vi "Logging Message Loop.vi"(8 "error in (no error)":errorcluster, 10 "Data Queue":refnum<queue>, 11 "Message Queues":T1) -> (0 "error out":errorcluster)   [LabVIEW 2021, in "Logging.lvlib"]
doc: "Message loop for handling messages pertaining to logging data."
uses:
  Logging.lvlib
  support/Message Queue/All Message Queues.ctl
  support/Message Queue/Message Cluster.ctl
  Acquisition/Acquired Data.ctl
  Logging State.ctl
  support/Message Queue/Enqueue Message (Single).vi
  <vilib>/Utility/error.llb/Error Cluster From Error Code.vi
  <vilib>/ErrorRing/Error Ring.xnode
  support/Message Queue/Message Queue.lvlib
  Settings/Settings.lvlib
  Acquisition/Acquisition.lvlib
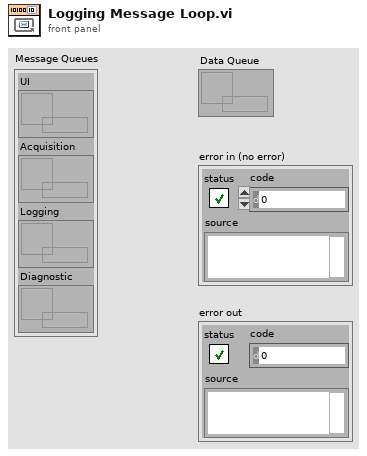
[diagram p1: front panel]
types:
  T1 = typedef "Message Queue.lvlib/All Message Queues.ctl" = cluster{"UI":refnum<queue>, "Acquisition":refnum<queue>, "Logging":refnum<queue>, "Diagnostic":refnum<queue>}
  T2 = typedef "Logging.lvlib/Logging State.ctl" = enum16{"Idle", "Logging"}
  T3 = typedef "Settings.lvlib/Settings.ctl" = cluster{"IO":T4, "Log":T11, "Debug":T13}
  T4 = typedef "Acquisition.lvlib/Hardware Configuration.ctl" = cluster{"Channel Settings":T5[], "Sensor Intervals":T7[], "Sensor Token":T9, "API":T10}
  T5 = typedef "Acquisition.lvlib/Channel Settings.ctl" = cluster{"Name":string, "Terminal Information":cluster{"IO Device":T6, "Channel Number":i32}, "Calibration Information":cluster{"Excitation Voltage":dbl, "Calibration Factor":dbl, "Zero Value":dbl, "Calibration Formula":string}}
  T6 = typedef "Acquisition.lvlib/IO Device.ctl" = enum16{"none", "9219", "9401"}
  T7 = typedef "Interval Timer.lvlib/Repeat Interval.ctl" = cluster{"Interval":T8, "Count":i32}
  T8 = typedef "Interval Timer.lvlib/Interval Length.ctl" = enum16{"Manual control", "1 second", "10 seconds", "30 seconds", "60 seconds", "600 seconds", "1200 seconds", "3600 seconds"}
  T9 = typedef "Interval Timer.lvlib/Interval Token.ctl" = cluster{"Next reading in ms":u32, "Interval Index":i32, "Interval Occurrence":i32}
  T10 = typedef "Acquisition.lvlib/IO API.ctl" = enum16{"Simulated", "DAQmx"}
  T11 = typedef "Logging.lvlib/Logging Configuration.ctl" = cluster{"Path":path, "Spreadsheet":refnum<file>, "Mode":T12}
  T12 = typedef "Logging.lvlib/Logging Mode.ctl" = enum16{"Overwrite", "Append", "Create New"}
  T13 = typedef "Diagnostics.lvlib/Diagnostics Configuration.ctl" = cluster{"Messages":refnum<file>}
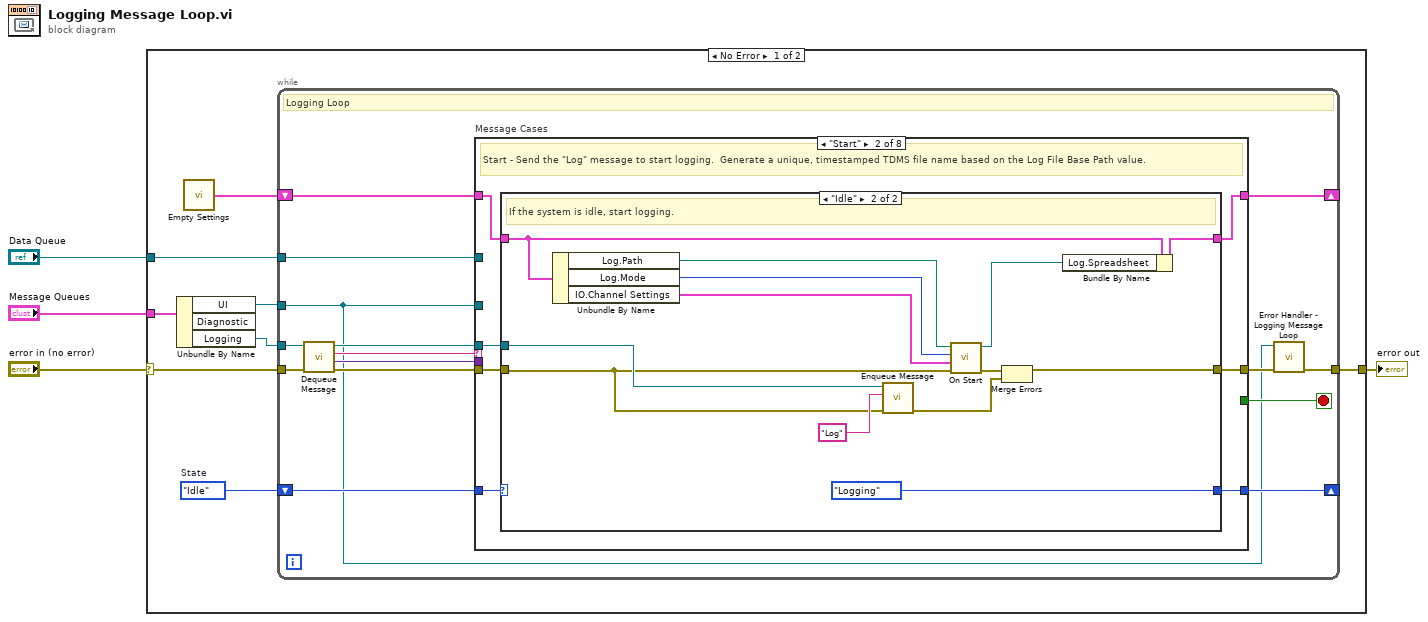
[diagram p0: block diagram]
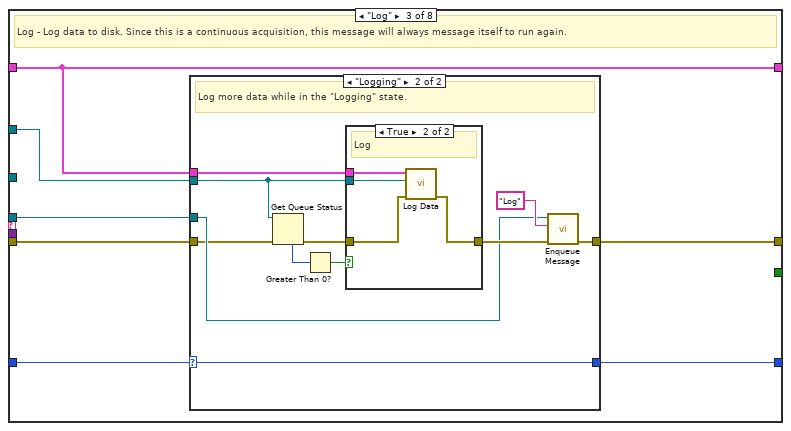
[diagram p4: hidden frame]
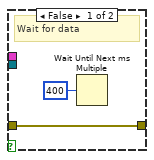
[diagram p6: hidden frame]
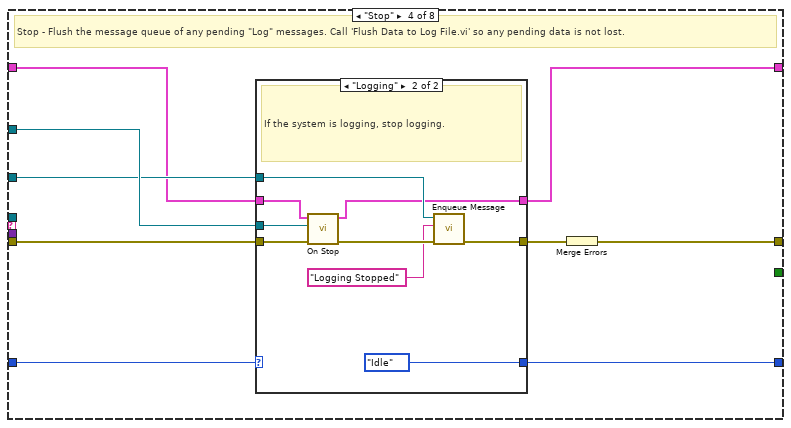
[diagram p7: hidden frame]
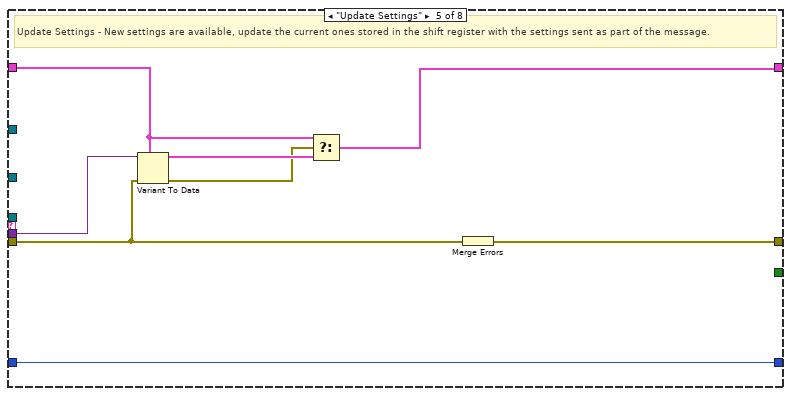
[diagram p9: hidden frame]
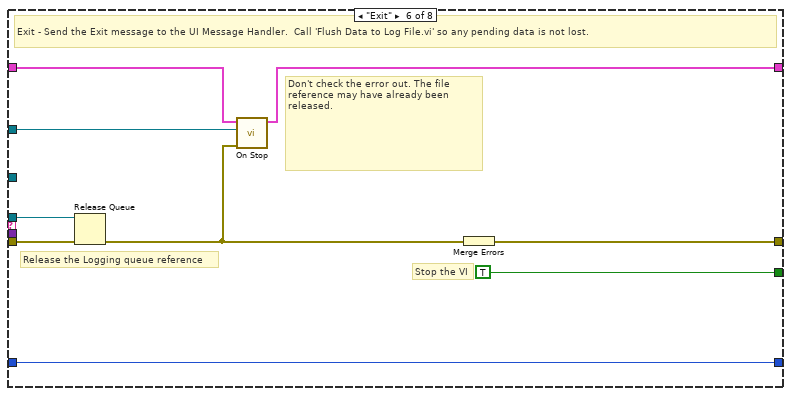
[diagram p10: hidden frame]
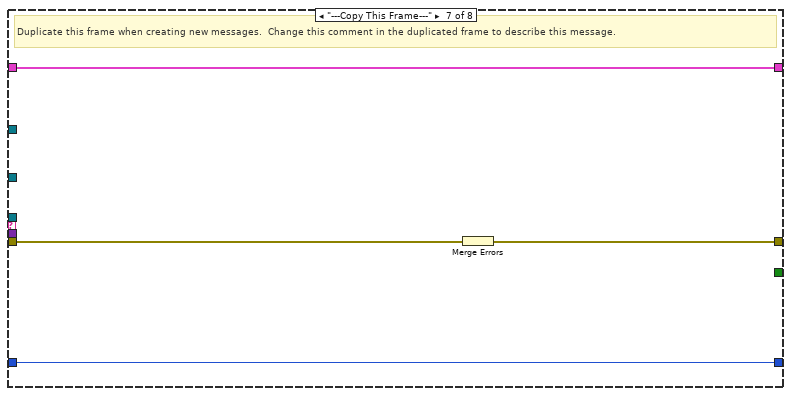
[diagram p11: hidden frame]
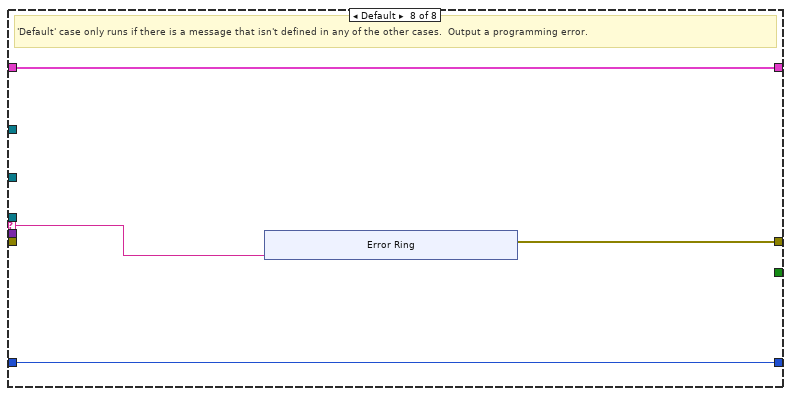
[diagram p12: hidden frame]
diagram:
  n1 = case shown="No Error" "error in (no error)" {
    selector: "error in (no error)" -> [w10 w133]
    tunnel: "Message Queues" -> [w12 _]
    tunnel: [w11 w133] -> w3
    tunnel: "Data Queue" -> [w9 _]
    frame No Error {
      w7 = Logging_State."Idle"  # State
      n2 = Unbundle By Name(w12) -> ("UI"=w8:refnum<queue>, "Logging"=w5:refnum<queue>)  [unwired: 1 out]
      n3 = call "Empty Settings.vi"() -> ("Settings"=w6:T3)
      n4 = while {
        tunnel: w5 -> [w19]
        shift-right: [w26] -> _
        shift-left: w6 -> [w27]
        tunnel: w8 -> [w13]
        tunnel: w9 -> [w18]
        shift-right: [w16] -> _
        shift-left: w7 -> [w17]
        tunnel: w10 -> [w24]
        tunnel: [w15] -> w11
        stop <- w25 stop-if-true
        # "Logging Loop"
        n5 = call "Dequeue Message.vi"("error in (no error)"=w24, "Message Queue"=w19) -> ("error out"=w23:errorcluster, "Message Data"=w21:variant, "Message"=w22:string, "dup Message Queue"=w20:refnum<queue>)  [unwired: 6 in]
        n6 = case "Message Cases" shown="\"Start\"" w22 {
          selector: w22 -> [_ _ _ _ _ _ _ w122]
          tunnel: w20 -> [_ w36 w59 _ _ w114 _ _]
          tunnel: w23 -> [w29 w35 w57 w85 w102 w115 w121 _]
          tunnel: [w29 w37 w60 w88 w108 w116 w119 w123] -> w14
          tunnel: w27 -> [w30 w34 w56 w80 w106 w110 w120 w125]
          tunnel: [w30 w33 w56 w81 w103 w109 w120 w125] -> w26
          tunnel: [_ _ _ _ _ TRUE _ _] -> w25
          tunnel: w21 -> [_ _ _ _ w107 _ _ _]
          tunnel: w13 -> [_ _ _ w82 _ _ _ _]
          tunnel: w18 -> [_ _ w58 w86 _ w112 _ _]
          tunnel: w17 -> [w28 w32 w55 w84 w101 w111 w118 w124]
          tunnel: [w28 w31 w54 w83 w101 w111 w118 w124] -> w16
          frame "Initialize" {
            # "Initialize - gets called when first launched. Currently a no-op."
          }
          frame "Start" {
            # "Start - Send the \"Log\" message to start logging.  Generate a unique, timestamped TDMS file name based on the Log File Base Path value."
            n7 = case shown="\"Idle\"" w32 {
              selector: w32 -> [w39 _]
              tunnel: [w38 w47] -> w37
              tunnel: w36 -> [_ w48]
              tunnel: w35 -> [w38 w46]
              tunnel: w34 -> [w40 w49]
              tunnel: [w40 w51] -> w33
              tunnel: [w39 Logging_State."Logging" ("State")] -> w31
              frame "Logging" {
                # "The system is already logging. Ignore the \"Start\" message."
              }
              frame "Idle" {
                # "If the system is idle, start logging."
                n8 = Unbundle By Name(w49) -> ("Log.Path"=w43:path, "Log.Mode"=w44:T12, "IO.Channel Settings"=w41:T5[])
                n9 = call-poly "Enqueue Message.vi"("error in (no error)"=w46, "Message"="Log", "Message Queue"=w48) -> ("error out"=w52:errorcluster)  [unwired: 7 in, 1 out]
                n10 = call "On Start.vi"("error in"=w46, "Channel Settings"=w41, "Mode"=w44, "file path"=w43) -> ("error out"=w45:errorcluster, "file reference"=w42:refnum<file>)  [unwired: 6 in]
                n11 = Merge Errors(w45, w52) -> (w47:errorcluster)
                n12 = Bundle By Name(cluster=w49, "Log.Spreadsheet"=w42) -> (w51:T3)
              }
            }
          }
          frame "Log" {
            # "Log - Log data to disk. Since this is a continuous acquisition, this message will always message itself to run again."
            n13 = case shown="\"Logging\"" w55 {
              selector: w55 -> [w62 w71]
              tunnel: [w61 w70] -> w60
              tunnel: w59 -> [_ w68]
              tunnel: w58 -> [_ w65]
              tunnel: w57 -> [w61 w67]
              tunnel: w56 -> [_ w72]
              tunnel: [w62 w71] -> w54
              frame "Idle" {
                # "Ignore \"Log\" messages when the logging is idle."
              }
              frame "Logging" {
                # "Log more data while in the \"Logging\" state."
                n14 = Get Queue Status(queue=w65, error in (no error)=w67) -> (error out=w66:errorcluster, # elements in queue=w64:i32)  [unwired: 1 in, 6 out]
                n15 = Greater Than 0?(x=w64) -> (x > 0?=w63:bool)
                n16 = case shown="True" w63 {
                  tunnel: w65 -> [_ w79]
                  tunnel: w72 -> [_ w78]
                  tunnel: w66 -> [w75 w77]
                  tunnel: [w75 w76] -> w69
                  frame False {
                    # "Wait for data"
                    n17 = Wait Until Next ms Multiple(millisecond multiple=u32 400) -> ()  [unwired: 1 out]
                  }
                  frame True {
                    # "Log"
                    n18 = call "Log Data.vi"("error in (no error)"=w77, "Data Queue"=w79, "Settings"=w78) -> ("error out"=w76:errorcluster)  [unwired: 8 in]
                  }
                }
                n19 = call-poly "Enqueue Message.vi"("error in (no error)"=w69, "Message"="Log", "Message Queue"=w68) -> ("error out"=w70:errorcluster)  [unwired: 7 in, 1 out]
              }
            }
          }
          frame "Stop" {
            # "Stop - Flush the message queue of any pending \"Log\" messages. Call 'Flush Data to Log File.vi' so any pending data is not lost."
            n20 = case shown="\"Logging\"" w84 {
              selector: w84 -> [w90 _]
              tunnel: [w91 w95] -> w87
              tunnel: w86 -> [_ w99]
              tunnel: w80 -> [w89 w98]
              tunnel: w85 -> [w91 w97]
              tunnel: [w90 Logging_State."Idle" ("State")] -> w83
              tunnel: w82 -> [_ w94]
              tunnel: [w89 w92] -> w81
              frame "Idle" {
                # "The system is already idle. Ignore the \"Stop\" message."
              }
              frame "Logging" {
                # "If the system is logging, stop logging."
                n21 = call "On Stop.vi"("error in (no error)"=w97, "Data Queue"=w99, "Settings in"=w98) -> ("error out"=w100:errorcluster, "Settings out"=w92:T3)  [unwired: 7 in]
                n22 = call-poly "Enqueue Message.vi"("error in (no error)"=w100, "Message"="Logging Stopped", "Message Queue"=w94) -> ("error out"=w95:errorcluster)  [unwired: 7 in, 1 out]
              }
            }
            n23 = Merge Errors(w87) -> (w88:errorcluster)
          }
          frame "Update Settings" {
            # "Update Settings - New settings are available, update the current ones stored in the shift register with the settings sent as part of the message."
            n24 = Variant To Data(error in=w102, type=w106, Variant=w107) -> (data=w105:T3, error out=w104:errorcluster)
            n25 = Select(t=w106, s=w104, f=w105) -> (s? t:f=w103:T3)
            n26 = Merge Errors(w102) -> (w108:errorcluster)
          }
          frame "Exit" {
            # "Don't check the error out. The file reference may have already been released."
            # "Release the Logging queue reference"
            # "Stop the VI"
            # "Exit - Send the Exit message to the UI Message Handler.  Call 'Flush Data to Log File.vi' so any pending data is not lost."
            n27 = Release Queue(queue=w114, error in (no error)=w115) -> (error out=w113:errorcluster)  [unwired: 1 in, 2 out]
            n28 = call "On Stop.vi"("error in (no error)"=w113, "Data Queue"=w112, "Settings in"=w110) -> ("Settings out"=w109:T3)  [unwired: 7 in, 1 out]
            n29 = Merge Errors(w113) -> (w116:errorcluster)
          }
          frame "---Copy This Frame---" {
            # "Duplicate this frame when creating new messages.  Change this comment in the duplicated frame to describe this message."
            n30 = Merge Errors(w121) -> (w119:errorcluster)
          }
          frame Default {
            # "'Default' case only runs if there is a message that isn't defined in any of the other cases.  Output a programming error."
            n31 = xnode "Error Ring"("parameter 0"=w122) -> ("error out"=w123:errorcluster)
          }
        }
        n32 = call "Error Handler - Logging Message Loop.vi"("error in (no error)"=w14, "Message Queue"=w13) -> ("dup error in"=w15:errorcluster)  [unwired: 8 in, 1 out]
      }
    }
    frame Error {
    }
  }
  "error out" <- w3
